vi "ProgressWindowDialog.vi"(0 "ReferenceIn":refnum<class "ClassWriter.lvclass">, 5 "error in (no error)":errorcluster) -> (19 "error out":errorcluster)   [LabVIEW 2020, in "ClassWriter.lvclass"]
uses:
  ClassWriter.lvclass
  <vilib>/picture/picture.llb/imagedata.ctl
  ClassWriter.lvclass/ClassWriter.ctl
panel:
  out "Message":string
  out "Bar":picture
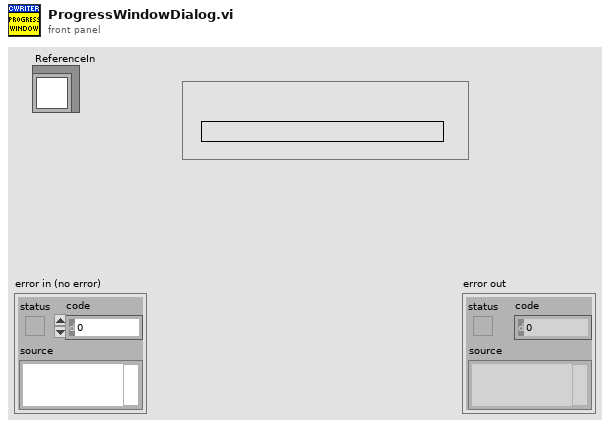
[diagram p1: front panel]
types:
  T1 = typedef "imagedata.ctl" = cluster{"image type":i32, "image depth":i32, "image":u8[], "mask":u8[], "colors":u32[], "Rectangle":cluster{"left":i16, "top":i16, "right":i16, "bottom":i16}}
  T2 = cluster{"i":i32, "end":i32, "Right":bool, "Event":refnum<event-registration>}
  T3 = enum32{"Invalid", "Default", "Floating", "Floating/Auto-Hide", "Modal"}
  T4 = cluster{"left":i16, "top":i16, "right":i16, "bottom":i16}
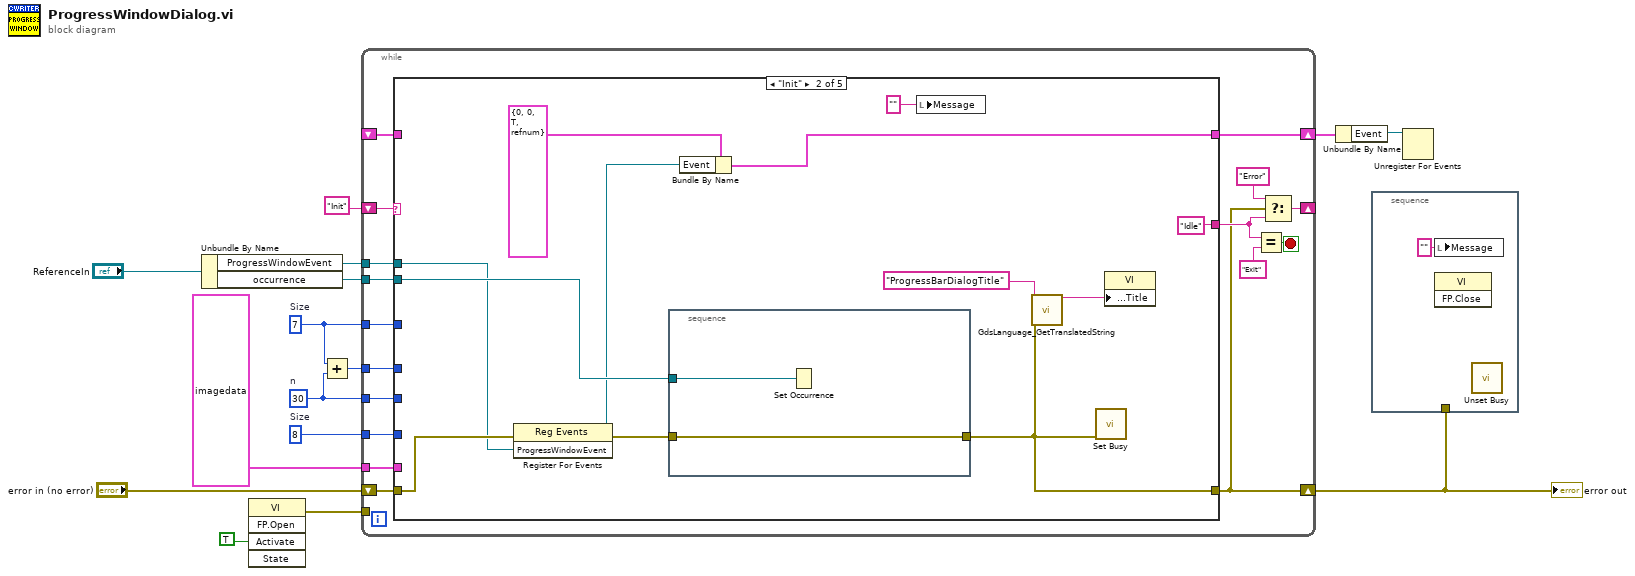
[diagram p0: block diagram]
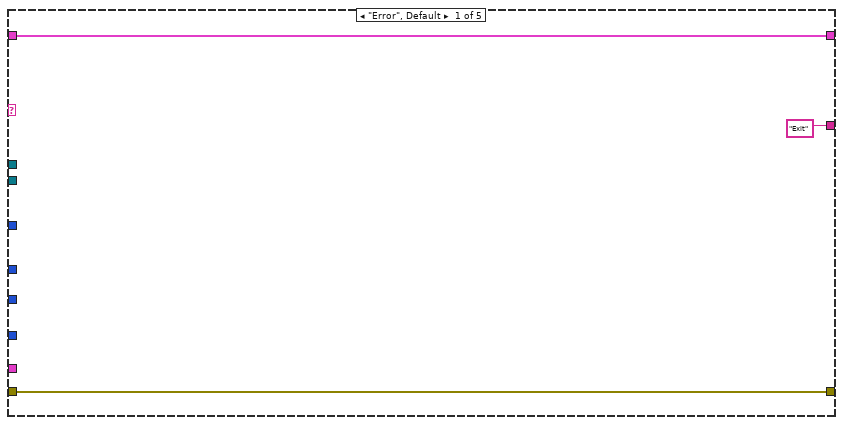
[diagram p2: hidden frame]
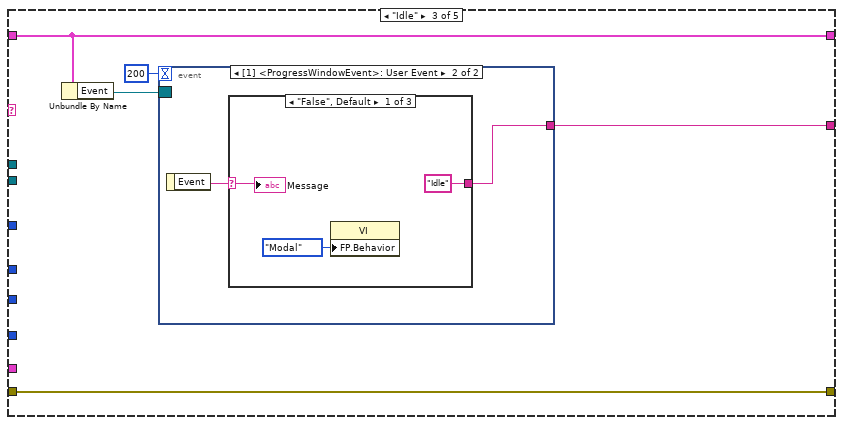
[diagram p3: hidden frame]
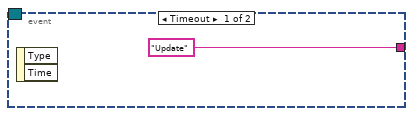
[diagram p4: hidden frame]
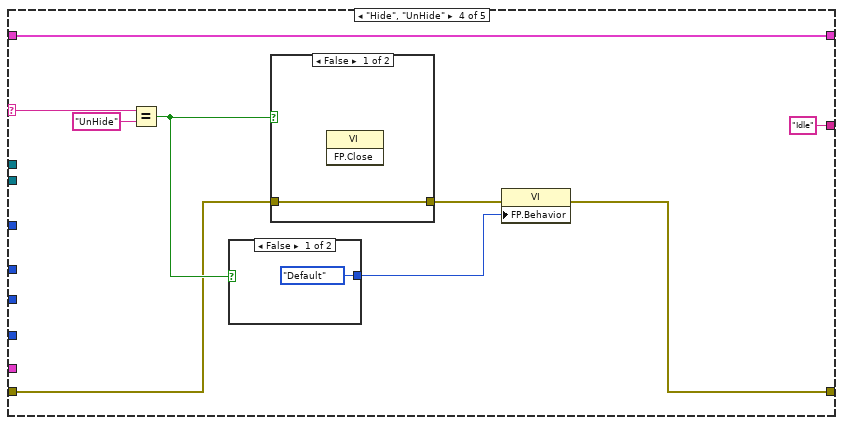
[diagram p7: hidden frame]
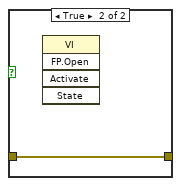
[diagram p8: hidden frame]
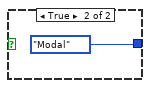
[diagram p9: hidden frame]
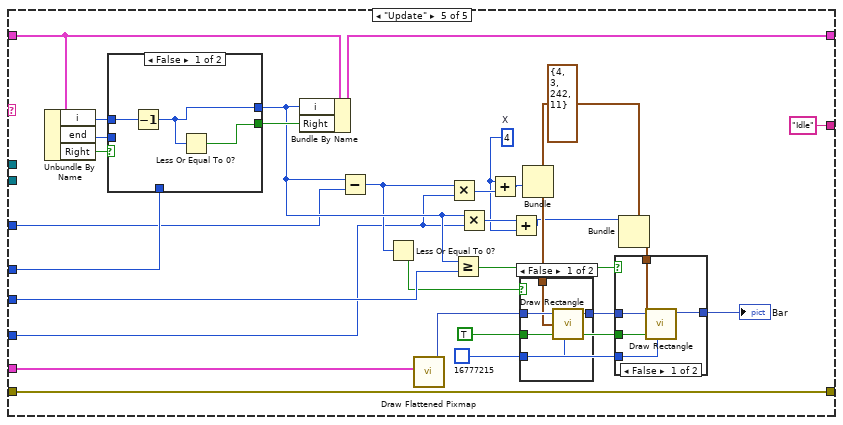
[diagram p10: hidden frame]
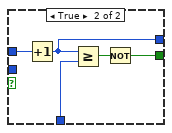
[diagram p13: hidden frame]
diagram:
  w8 = 7  # Size
  w9 = 8  # Size
  w7 = 30  # n
  n1 = Unbundle By Name("ReferenceIn") -> ("ProgressWindowEvent"=w13:refnum<user-event>, "occurrence"=w10:refnum<k4>)
  n2 = invoke class="VI" method="FP.Open"("Activate"=TRUE ("Front Panel Window:Open")) -> (error out=w2:errorcluster)  [unwired: 4 in, 4 out]
  n3 = Add(x=w8, y=w7) -> (x+y=w6:i32)
  n4 = while {
    shift-right: [w25] -> w4
    shift-left: "error in (no error)" -> [w32]
    shift-right: [w30] -> _
    shift-left: "Init" -> [w31]
    shift-right: [w24] -> w12
    shift-left: _ -> [w23]
    tunnel: w13 -> [w22]
    tunnel: w10 -> [w21]
    tunnel: w9 -> [w20]
    tunnel: w7 -> [w19]
    tunnel: w8 -> [w18]
    tunnel: T1 {"image type"=0, "image depth"=24, "image"=array[9555 elements], "mask"=[], "colors"=[], "Rectangle"={"left"=0, "top"=0, "right"=245, "bottom"=13}} ("image data") -> [w17]
    tunnel: w6 -> [w16]
    tunnel: w2 -> [_]
    stop <- w29 stop-if-true
    n5 = case shown="\"Init\"" w31 {
      selector: w31 -> [_ _ _ w70 _]
      tunnel: w32 -> [w35 w43 w52 w63 w105]
      tunnel: [w35 w37 w52 w66 w105] -> w25
      tunnel: ["Exit" "Idle" w50 "Idle" ("f") "Idle"] -> w26
      tunnel: [w33 w45 w54 w71 w86] -> w24
      tunnel: w23 -> [w33 _ w54 w71 w89]
      tunnel: w22 -> [_ w41 _ _ _]
      tunnel: w21 -> [_ w42 _ _ _]
      tunnel: w20 -> [_ _ _ _ w79]
      tunnel: w19 -> [_ _ _ _ w88]
      tunnel: w18 -> [_ _ _ _ w84]
      tunnel: w17 -> [_ _ _ _ w100]
      tunnel: w16 -> [_ _ _ _ w91]
      frame "Error", Default {
      }
      frame "Init" {
        n6 = register-events(error in=w43, w41) -> (reference out=w40:refnum<event-registration>, error out=w44:errorcluster)  [unwired: 1 in]
        n7 = stacked-sequence {
          tunnel: w44 -> [w49]
          tunnel: [w49] -> w37
          tunnel: w42 -> [w48]
          frame #0 {
            n8 = Set Occurrence(w48) -> ()
          }
        }
        n9 = Bundle By Name(cluster=T2 {"i"=0, "end"=0, "Right"=TRUE, "Event"=refnum}, "Event"=w40) -> (w45:T2)
        n10 = local write "Message"("" ("Message")) -> ()
        n11 = call "GdsLanguage_GetTranslatedString.vi"("StringID(s)"="ProgressBarDialogTitle", "error in (no error)"=w37) -> ("FirstStringOut"=w38:string)  [unwired: 14 in, 3 out]
        n12 = call <vilib>:"Set Busy.vi"("error in (no error)"=w37) -> ()  [unwired: 9 in, 2 out]
        n13 = property class="VI"("Front Panel.Title"=w38) -> ()  [unwired: 2 in, 2 out]
      }
      frame "Idle" {
        n14 = Unbundle By Name(w54) -> ("Event"=w53:refnum<event-registration>)
        n15 = event shown="[1] <ProgressWindowEvent>: User Event" {
          selector: w53 -> [_ _]
          dyn-events: _ -> [_ _]
          timeout: 200 -> [_ _]
          tunnel: ["Update" w56] -> w50
          event Timeout {
            n16 = event-data() -> ()  [unwired: 1 in, 2 out]
          }
          event User Event {
            n17 = event-data() -> ("Event"=w57:string)  [unwired: 1 in]
            n18 = case shown="\"False\", Default" w57 {
              selector: w57 -> [w60 w61 w62]
              tunnel: ["Idle" ("f") w61 w62] -> w56
              frame "False", Default {
                n19 = property class="VI"("FP.Behavior"=T3."Modal" ("Front Panel Window:Behavior")) -> ()  [unwired: 2 in, 2 out]
                "Message" <- w60
              }
              frame "Exit" {
              }
              frame "Hide", "UnHide" {
              }
            }
          }
        }
      }
      frame "Hide", "UnHide" {
        n20 = Equal?(x=w70, y="UnHide") -> (x = y?=w65:bool)
        n21 = case shown="False" w65 {
          tunnel: [T3."Default" ("Front Panel Window:Behavior") T3."Modal" ("Front Panel Window:Behavior")] -> w67
          frame False {
          }
          frame True {
          }
        }
        n22 = case shown="False" w65 {
          tunnel: [w72 w73] -> w64
          tunnel: w63 -> [w72 w73]
          frame False {
            n23 = invoke class="VI" method="FP.Close"() -> ()  [unwired: 3 in, 3 out]
          }
          frame True {
            n24 = invoke class="VI" method="FP.Open"() -> ()  [unwired: 5 in, 5 out]
          }
        }
        n25 = property class="VI"(error in=w64, "FP.Behavior"=w67) -> (error out=w66:errorcluster)  [unwired: 1 in, 1 out]
      }
      frame "Update" {
        w96 = T4 {"left"=4, "top"=3, "right"=242, "bottom"=11} ("rect")
        w77 = 4  # X
        w94 = u32 16777215 ("color(black)")
        w93 = TRUE ("fill?(F)")
        n26 = Unbundle By Name(w89) -> ("i"=w101:i32, "end"=w102:i32, "Right"=w103:bool)
        n27 = case shown="False" w103 {
          tunnel: w102 -> [_ _]
          tunnel: w101 -> [w120 w125]
          tunnel: w91 -> [_ w124]
          tunnel: [w118 w122] -> w90
          tunnel: [w119 w121] -> w85
          frame False {
            n28 = Decrement(x=w120) -> (x-1=w119:i32)
            n29 = Less Or Equal To 0?(x=w119) -> (x <= 0?=w118:bool)
          }
          frame True {
            n30 = Increment(x=w125) -> (x+1=w121:i32)
            n31 = Greater Or Equal?(x=w121, y=w124) -> (x >= y?=w123:bool)
            n32 = Not(x=w123) -> (.not. x?=w122:bool)
          }
        }
        n33 = Bundle By Name(cluster=w89, "i"=w85, "Right"=w90) -> (w86:T2)
        n34 = Subtract(x=w85, y=w84) -> (x-y=w80:i32)
        n35 = Less Or Equal To 0?(x=w80) -> (x <= 0?=w83:bool)
        n36 = call <vilib>:"Draw Flattened Pixmap.vi"("image data"=w100) -> ("new picture"=w99:picture)  [unwired: 8 in]
        n37 = Multiply(x=w80, y=w79) -> (x*y=w78:i32)
        n38 = Greater Or Equal?(x=w85, y=w88) -> (x >= y?=w87:bool)
        n39 = Multiply(x=w85, y=w79) -> (x*y=w82:i32)
        n40 = Add(x=w77, y=w78) -> (x+y=w76:i32)
        n41 = Add(x=w82, y=w77) -> (x+y=w81:i32)
        n42 = Bundle(cluster=w96, "right"=w76) -> (w98:T4)  [unwired: 3 in]
        n43 = case shown="False" w83 {
          tunnel: w99 -> [w110 w111]
          tunnel: w98 -> [w109 _]
          tunnel: [w108 w111] -> w97
          tunnel: w94 -> [w107 _]
          tunnel: w93 -> [w106 _]
          frame False {
            n44 = call <vilib>:"Draw Rectangle.vi"("picture"=w110, "rect"=w109, "fill?(F)"=w106, "color(black)"=w107) -> ("new picture"=w108:picture)  [unwired: 5 in]
          }
          frame True {
          }
        }
        n45 = Bundle(cluster=w96, "left"=w81) -> (w95:T4)  [unwired: 3 in]
        n46 = case shown="False" w87 {
          tunnel: w97 -> [w116 w117]
          tunnel: w95 -> [w115 _]
          tunnel: w94 -> [w114 _]
          tunnel: w93 -> [w113 _]
          tunnel: [w112 w117] -> w92
          frame False {
            n47 = call <vilib>:"Draw Rectangle.vi"("picture"=w116, "rect"=w115, "fill?(F)"=w113, "color(black)"=w114) -> ("new picture"=w112:picture)  [unwired: 5 in]
          }
          frame True {
          }
        }
        "Bar" <- w92
      }
    }
    n48 = Equal?(x=w26, y="Exit") -> (x = y?=w29:bool)
    n49 = Select(t="Error", s=w25, f=w26) -> (s? t:f=w30:string)
  }
  "error out" <- w4
  n50 = Unbundle By Name(w12) -> ("Event"=w11:refnum<event-registration>)
  n51 = stacked-sequence {
    tunnel: w4 -> [_]
    frame #0 {
      n52 = local write "Message"("" ("Message")) -> ()
      n53 = invoke class="VI" method="FP.Close"() -> ()  [unwired: 3 in, 3 out]
      n54 = call <vilib>:"Unset Busy.vi"() -> ()  [unwired: 11 in, 1 out]
    }
  }
  n55 = Unregister For Events(event registration refnum=w11) -> ()  [unwired: 1 in, 1 out]
